vi "OwnBuild20261013_CreateSDIST.vi"() -> ()   [LabVIEW 2024]
uses:
  <vilib>/AppBuilder/AB_API/SDIST/NI_AB_API_SDIST.lvclass
panel:
  out "error out":errorcluster caption="错误输出"
  in  "Save Project Path":path
  in  "Destination":path
  in  "Spec Name":string caption="程序生成规范名称"
  in  "Member ID":string
  in  "Project Path":path
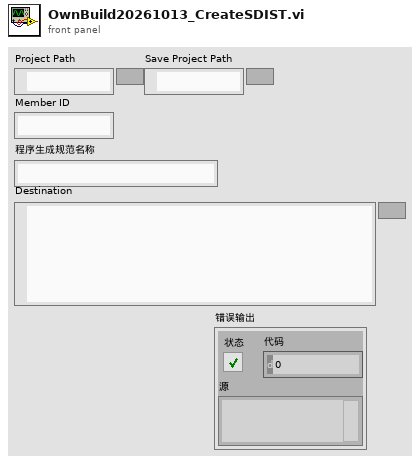
[diagram p1: front panel]
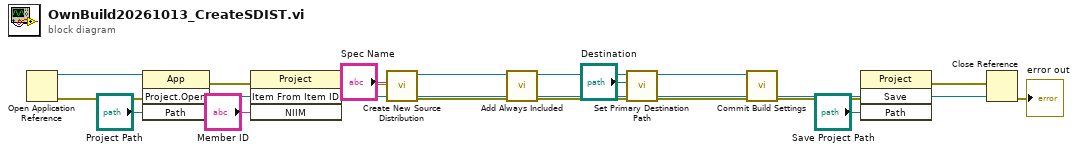
[diagram p0: block diagram]
diagram:
  n1 = Open Application Reference() -> (0:w18:errorcluster, 3:w20:refnum<vi>)  [unwired: 4 in]
  n2 = invoke class="App" method="Project.Open"(reference=w20, error in=w18, "Path"="Project Path") -> (error out=w15:errorcluster, "Project:Open"=w17:refnum<vi>)  [unwired: 1 in, 2 out]
  n3 = invoke class="Project" method="Item From Item ID"(reference=w17, error in=w15, "NIIM"="Member ID") -> (error out=w13:errorcluster, "GetItemFromNIIM"=w11:refnum<vi>)  [unwired: 1 in, 2 out]
  n4 = call <vilib>:"Create New Source Distribution.vi"("error in (no error)"=w13, "Build specification name"="Spec Name", "Project Refnum"=w17) -> ("error out"=w10:errorcluster, "SDIST out"=w12:refnum<class "NI_AB_API_SDIST.lvclass">)  [unwired: 7 in]
  n5 = call-dynamic "Add Always Included.vi"("error in (no error)"=w10, "ProjectItem Refnum"=w11, "SDIST in"=w12) -> ("error out"=w7:errorcluster, "SDIST out"=w9:refnum<class "NI_AB_API_SDIST.lvclass">)  [unwired: 7 in]
  n6 = call-dynamic "Set Primary Destination Path.vi"("error in (no error)"=w7, "Destination path"="Destination", "Build in"=w9) -> ("error out"=w5:errorcluster, "Build out"=w6:refnum<class "NI_AB_API_SDIST.lvclass">)  [unwired: 7 in]
  n7 = call-dynamic "Commit Build Settings.vi"("error in (no error)"=w5, "SDIST in"=w6) -> ("error out"=w3:errorcluster)  [unwired: 8 in, 1 out]
  n8 = invoke class="Project" method="Save"(reference=w17, error in=w3, "Path"="Save Project Path") -> (error out=w2:errorcluster)  [unwired: 1 in, 3 out]
  n9 = Close Reference(reference=w17, error in (no error)=w2) -> (error out=→"error out":errorcluster)
